vi "RemoteVI Popup Click.vi"(0 "hWnd":u64, 1 "popup since":u32, 5 "posts":cluster{"msg":u32, "wParam":u64, "lParam":i64}[](array[cluster]), 7 "point":cluster{"x":i32, "y":i32}, 9 "windows":T1(array[cluster]), 11 "error in":errorcluster) -> (15 "error out":errorcluster)   [LabVIEW 2020, in "RemoteVI.lvlib"]
doc: "The popup branch of RemoteVI Post Input.vi - a remote mouse button message while a LabVIEW popup is open (docs\\architecture.md, Popups). The host cursor never moves. The LabVIEW menus are listed fresh (RemoteVI List Menus.vi, deepest first; menus are never moved, so their real place is the logical one) and the one under the clicked point is found (RemoteVI Point On Popup.vi). On a menu the click is done with KEYS (RemoteVI Menu Click.vi: close the submenus above with VK_LEFT, move the highlight with VK_DOWN / VK_UP, VK_RETURN; a button-up is dropped). When that window takes no keys (colour picker, line width popup), or the point lies on another popup of the server's list (windows - graph palette popups, drop-downs), the MOUSE path clicks it (RemoteVI Plain Popup Click.vi: only that window is moved under the cursor for the message and moved back). A point outside every popup: a button-down closes all popups with WM_CANCELMODE (RemoteVI Cancel Popups.vi), a button-up is dropped. No waiting beyond LabVIEW handling each key or message; no VI Server call."
uses:
  RemoteVI.lvlib
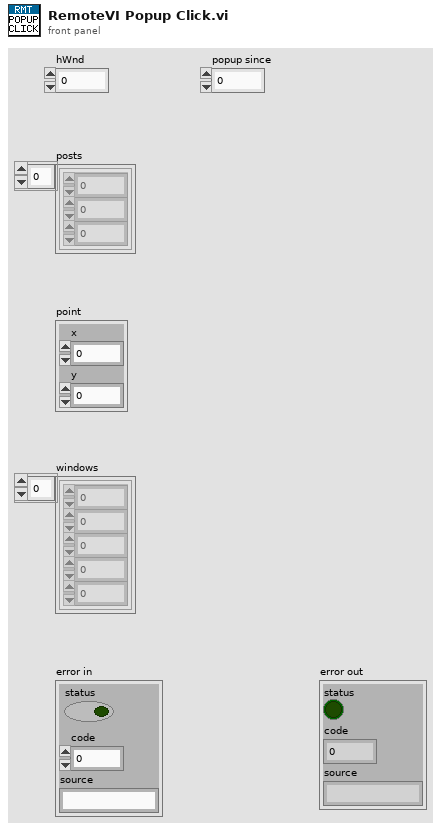
[diagram p1: front panel]
types:
  T1 = cluster{"hwnd":u64, "x":i32, "y":i32, "w":i32, "h":i32}[]
  T2 = cluster{"hwnd":u64, "x":i32, "y":i32, "w":i32, "h":i32}
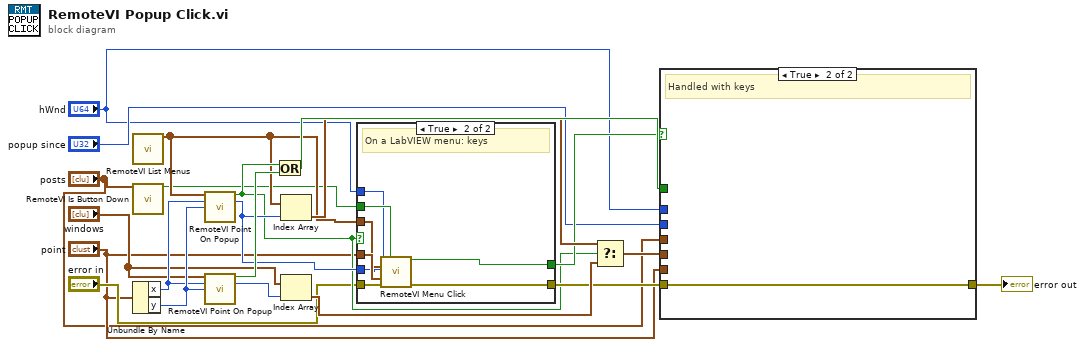
[diagram p0: block diagram]
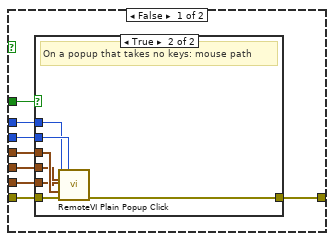
[diagram p2: hidden frame]
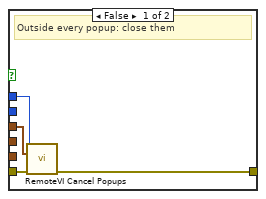
[diagram p3: hidden frame]
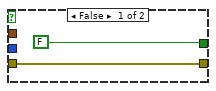
[diagram p4: hidden frame]
diagram:
  n1 = call "RemoteVI List Menus.vi"() -> ("menus"=w10:T1)  [unwired: 15 in]
  n2 = call "RemoteVI Is Button Down.vi"("posts"="posts") -> ("button down?"=w9:bool)  [unwired: 14 in]
  n3 = Unbundle By Name("point") -> ("x"=w7:i32, "y"=w8:i32)
  n4 = call "RemoteVI Point On Popup.vi"("windows"=w10, "x"=w7, "y"=w8) -> ("on popup?"=w11:bool, "index"=w12:i32)  [unwired: 11 in]
  n5 = call "RemoteVI Point On Popup.vi"("windows"="windows", "x"=w7, "y"=w8) -> ("on popup?"=w13:bool, "index"=w14:i32)  [unwired: 11 in]
  n6 = Or(x=w11, y=w13) -> (x .or. y?=w20:bool)
  n7 = Index Array(array=w10, index=w12) -> (element=w17:T2)
  n8 = Index Array(array="windows", index=w14) -> (element=w18:T2)
  n9 = case shown="True" w11 {
    tunnel: "error in" -> [w22 w24]
    tunnel: "hWnd" -> [_ w25]
    tunnel: "point" -> [_ w28]
    tunnel: w10 -> [_ w26]
    tunnel: w9 -> [_ w29]
    tunnel: w12 -> [_ w27]
    tunnel: [w22 w31] -> w15
    tunnel: [FALSE w30] -> w16
    frame False {
    }
    frame True {
      # "On a LabVIEW menu: keys"
      n10 = call "RemoteVI Menu Click.vi"("hWnd"=w25, "button down?"=w29, "menus"=w26, "k"=w27, "point"=w28, "error in"=w24) -> ("handled?"=w30:bool, "error out"=w31:errorcluster)  [unwired: 8 in]
    }
  }
  n11 = Select(t=w17, s=w11, f=w18) -> (s? t:f=w19:T2)
  n12 = case shown="True" w16 {
    tunnel: "hWnd" -> [w33 _]
    tunnel: "point" -> [w36 _]
    tunnel: "posts" -> [w37 _]
    tunnel: "popup since" -> [w38 _]
    tunnel: w20 -> [w34 _]
    tunnel: w19 -> [w35 _]
    tunnel: w15 -> [w32 w51]
    tunnel: [w39 w51] -> w21
    frame False {
      n13 = case shown="True" w34 {
        tunnel: w33 -> [w41 w45]
        tunnel: w36 -> [_ w47]
        tunnel: w37 -> [w42 w48]
        tunnel: w38 -> [_ w49]
        tunnel: w35 -> [_ w46]
        tunnel: w32 -> [w40 w44]
        tunnel: [w43 w50] -> w39
        frame False {
          # "Outside every popup: close them"
          n14 = call "RemoteVI Cancel Popups.vi"("hWnd"=w41, "posts"=w42, "error in"=w40) -> ("error out"=w43:errorcluster)  [unwired: 12 in]
        }
        frame True {
          # "On a popup that takes no keys: mouse path"
          n15 = call "RemoteVI Plain Popup Click.vi"("hWnd"=w45, "popup since"=w49, "window"=w46, "point"=w47, "posts"=w48, "error in"=w44) -> ("error out"=w50:errorcluster)  [unwired: 9 in]
        }
      }
    }
    frame True {
      # "Handled with keys"
    }
  }
  "error out" <- w21
